vi "Enqueue Command.vi"(4 "ack timeout (0 ms: no ack)":i32, 6 "query notifier":refnum<notifier>, 8 "error in (no error)":errorcluster, 9 "args":variant, 10 "command":string, 11 "ConfigManager.Text in":refnum<class "ConfigManager.Text.lvclass">) -> (0 "error out":errorcluster, 1 "Ack?":bool, 3 "ConfigManager.Text out":refnum<class "ConfigManager.Text.lvclass">)   [LabVIEW 2013, in "CfgManager.Text.lvlib" / "ConfigManager.Text.lvclass"]
uses:
  ConfigManager.Text.lvclass
  Response - cluster.ctl
  ConfigManager.Text.lvclass/ConfigManager.Text.ctl
  payload -- cluster.ctl
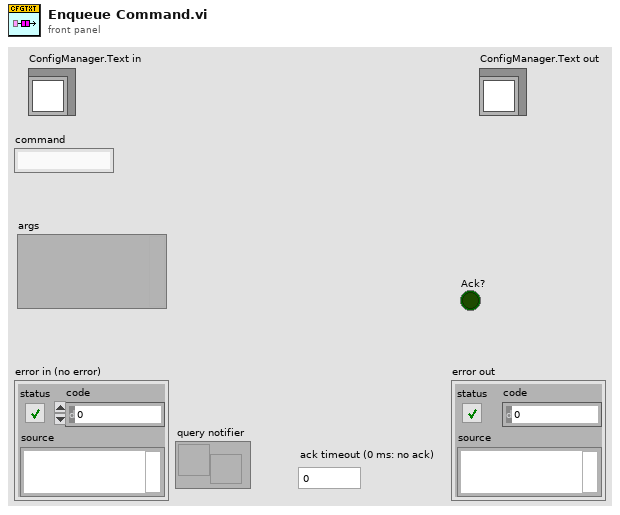
[diagram p1: front panel]
types:
  T1 = typedef "CfgManager.Text.lvlib/ConfigManager.Text.lvclass/payload -- cluster.ctl" = cluster{"command":string, "args":variant, "query":refnum<notifier>, "ack":refnum<notifier>}
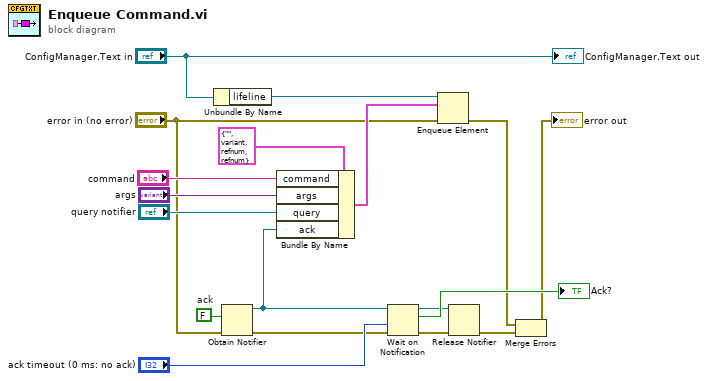
[diagram p0: block diagram]
diagram:
  w6 = FALSE  # ack
  n1 = Unbundle By Name("ConfigManager.Text in") -> ("lifeline"=w2:refnum<queue>)
  n2 = Obtain Notifier(notification data type=w6, error in (no error)="error in (no error)") -> (notifier out=w13:refnum<notifier>, error out=w5:errorcluster)  [unwired: 2 in, 1 out]
  n3 = Bundle By Name(cluster=T1 {"command"="", "args"=variant, "query"=refnum, "ack"=refnum} ("payload"), "command"="command", "args"="args", "query"="query notifier", "ack"=w13) -> (w18:T1)
  n4 = Wait on Notification(notifier=w13, timeout in ms (-1)="ack timeout (0 ms: no ack)", error in (no error)=w5) -> (notifier out=w4:refnum<notifier>, notification=→"Ack?":bool, error out=w3:errorcluster)  [unwired: 1 in, 1 out]
  n5 = Enqueue Element(queue=w2, element=w18, error in (no error)="error in (no error)") -> (error out=w9:errorcluster)  [unwired: 1 in, 2 out]
  n6 = Release Notifier(notifier=w4, error in (no error)=w3) -> (error out=w10:errorcluster)  [unwired: 1 in, 2 out]
  n7 = Merge Errors(w9, w10) -> (→"error out":errorcluster)
  "ConfigManager.Text out" <- "ConfigManager.Text in"
